vi "Tag Sample Valid.vi"(0 "Heartbeat":dbl, 1 "tx Degrees":dbl, 5 "Previous Heartbeat":dbl, 7 "Target Valid":dbl, 9 "Tag ID":dbl, 11 "error in (no error)":errorcluster) -> (4 "Valid Sample":bool, 15 "error out":errorcluster)   [LabVIEW 2025]
doc: "Accept only an AprilTag result from a new Limelight heartbeat: tv=1, tid>=1, finite tx within 35 degrees. Missing NT entries fail closed."
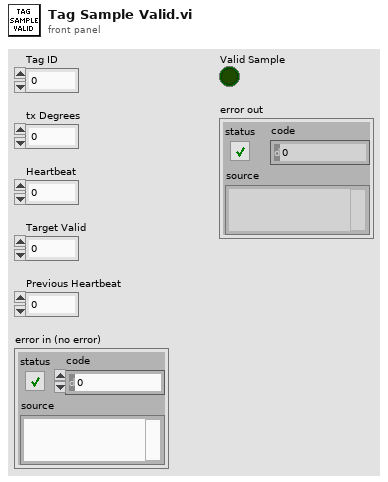
[diagram p1: front panel]
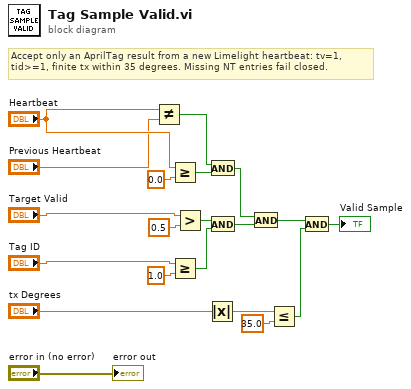
[diagram p0: block diagram]
diagram:
  # "Accept only an AprilTag result from a new Limelight heartbeat: tv=1,\ntid>=1, finite tx within 35 degrees. Missing NT entries fail closed."
  n1 = Not Equal?(x="Heartbeat", y="Previous Heartbeat") -> (x != y?=w10:bool)
  n2 = Greater Or Equal?(x="Heartbeat", y=0.0) -> (x >= y?=w9:bool)
  n3 = Greater Or Equal?(x="Tag ID", y=1.0) -> (x >= y?=w7:bool)
  n4 = Greater?(x="Target Valid", y=0.5) -> (0:w8:bool)
  n5 = Absolute Value(x="tx Degrees") -> (abs(x)=w11:dbl)
  n6 = And(x=w10, y=w9) -> (x .and. y?=w6:bool)
  n7 = And(x=w8, y=w7) -> (x .and. y?=w5:bool)
  n8 = And(x=w6, y=w5) -> (x .and. y?=w4:bool)
  n9 = Less Or Equal?(x=w11, y=35.0) -> (x <= y?=w3:bool)
  n10 = And(x=w4, y=w3) -> (x .and. y?=→"Valid Sample":bool)
  "error out" <- "error in (no error)"
